vi "CSM - Unregister Status Change.vi"(0 "CSM Name":string, 5 "Source CSM Name (* as Default)":string="*", 7 "Status":string, 9 "Response Message (\"*\" as Default)":string="*", 11 "Error In":errorcluster caption="error in (no error)") -> (4 "CSM Name (Dup)":string, 15 "error out":errorcluster)   [LabVIEW 2017, in "Communicable State Machine.lvlib"]
doc: "This VI is obsolete. Please use `CSM - Unregister Broadcast.vi`\n\n## CSM - Unregister Broadcast.vi\nUnregister notifications of state changes from other CSM modules.\n\nIn Worker Mode and Chain of Responsibility Mode, the input node name is automatically parsed as the module name because CSM implements registrations on a per-module basis.\n\n<b>Reference Example</b>: `2. Caller is CSM Scenario\\CSM Example - Caller is a CSM.vi`.\n\n> - Ref: CSM Registration\n\n-- <b>Controls</b> --\n- <b>CSM Name</b>: CSM module name.\n- <b>Source CSM Name (* as Default)</b>: The CSM module generating the status. You can use `*` to represent all modules generating the same status.\n- <b>Trigger</b>: Trigger string.\n- <b>API (\"*\" as Default)</b>: The API name to unregister. If empty, it applies to all APIs.\n\n-- <b>Indicators</b> --\n- <b>CSM Name (Dup)</b>: A copy of the input CSM module name."
uses:
  Communicable State Machine.lvlib
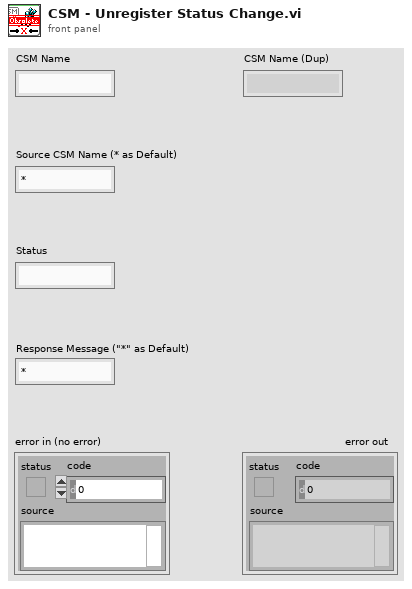
[diagram p1: front panel]
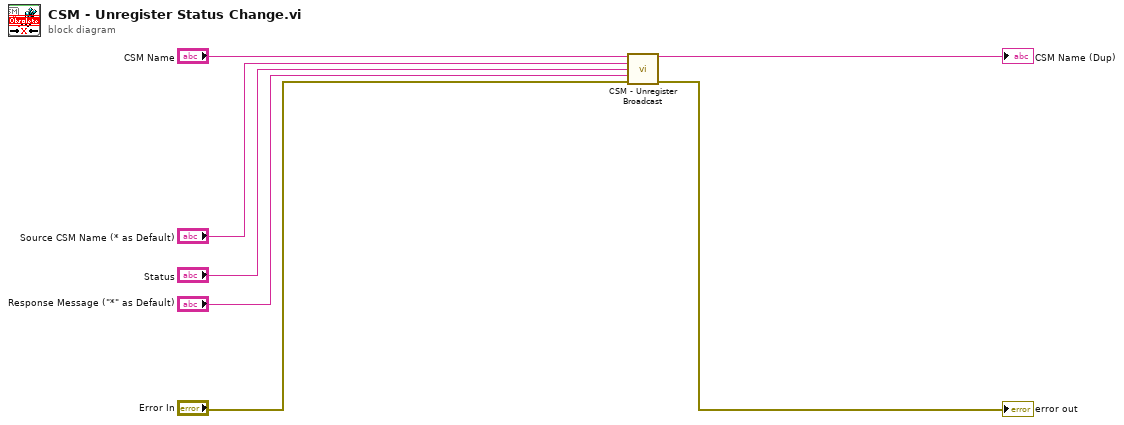
[diagram p0: block diagram]
diagram:
  n1 = call "CSM - Unregister Broadcast.vi"("CSM Name(Empty for Broadcast Event)"="CSM Name", "Source CSM Name (* as Default)"="Source CSM Name (* as Default)", "Trigger"="Status", "API (\"*\" as Default)"="Response Message (\"*\" as Default)", "Error In"="Error In") -> ("CSM Name (Dup)"=→"CSM Name (Dup)":string, "error out"=→"error out":errorcluster)  [unwired: 9 in]
